vi "Write Scalar Data.vi"(8 "error in (no error)":errorcluster, 9 "Changed?":bool[](array[boolean]), 10 "Values":dbl[](array[numeric]), 11 "Cluster":T1={"Name"="", "Data Type"=enum."<Null>", "session"=0, "Scalar Type"=enum."Standard", "Index"=0, "Length"=0, "attributes"=variant(refnum<k20> refnum), "default value"=variant(refnum<k20> refnum), "RegisterOffset"=0} {"Data Type" format="%.0x"}) -> (0 "error out":errorcluster, 2 "Values":dbl[](array[numeric]))   [LabVIEW 2020, in "FPGA Addon Engine.lvlib"]
uses:
  FPGA Addon Engine.lvlib
  APIs/FPGA Register IO/FPGA Register IO.lvlib
  3b4273db-2eef-454f-a9d7-15a0de1766a4.vi
  da3bfa8f-65e5-4f9a-8452-ca9305b9cf8c.vi
  e9b7ddae-4913-4a74-863a-ac6ad604f706.vi
  60e5d900-6671-49dd-bad3-679abba4dde3.vi
  4f31f09a-b0d0-4122-a737-4d514c13b382.vi
  857dc57c-d282-49ae-bb9f-12b46c14a078.vi
  77a28002-65ef-4437-82ec-1e91d7167048.vi
  660156fa-3609-4cbc-a785-e17faca41079.vi
  <vilib>/fxp/LVFixedPointRepRangeTypeDef.ctl
  <vilib>/fxp/LVFixedPointRepBitsTypeDef.ctl
  APIs/FPGA Register IO/TypeDefs/FXP Configuration.ctl
  Submodules/Source/Types/PWM.Measure.Digital.Settings.ctl
  Submodules/Source/Types/PWM.Measure.Analog.Settings.ctl
  Submodules/Source/Types/WSS.Generate.Digital.Settings.ctl
  Submodules/Source/Types/Sine.Generate.Settings.ctl
  Submodules/Source/Types/Static.Measure.Digital.Settings.ctl
  Submodules/Source/Types/Static.Generate.Digital.Settings.ctl
  Submodules/Source/Types/QuadratureEncoder.Measure.Digital.Settings.ctl
  Submodules/Source/Types/PWM.Generate.Digital.Settings.ctl
  APIs/FPGA Register IO/Write Methods/Write Data Register/Instances/Write SGL.vi
  APIs/FPGA Register IO/Write Methods/Write Data Register/Instances/Write U64.vi
  APIs/FPGA Register IO/Write Methods/Write Data Register/Instances/Write I32.vi
  APIs/FPGA Register IO/Write Methods/Write Data Register/Instances/Write I64.vi
  APIs/FPGA Register IO/Write Methods/Write Data Register/Instances/Write I16.vi
  APIs/FPGA Register IO/Write Methods/Write Data Register/Instances/Write U16.vi
  APIs/FPGA Register IO/Write Methods/Write Data Register/Instances/Write Boolean.vi
  APIs/FPGA Register IO/Write Methods/Write Data Register/Instances/Write FXP.vi
  APIs/FPGA Register IO/Write Methods/Write Data Register/Instances/Write I8.vi
  APIs/FPGA Register IO/Write Methods/Write Data Register/Instances/Write U8.vi
  APIs/FPGA Register IO/Write Methods/Write Data Register/Instances/Write U32.vi
  Types/Register Settings.ctl
  Addon Shared/Types/Scalar Type.ctl
  Addon Shared/FPGA Addon Shared.lvlib
  Addon Shared/Types/FPGA Addon Data Type.ctl
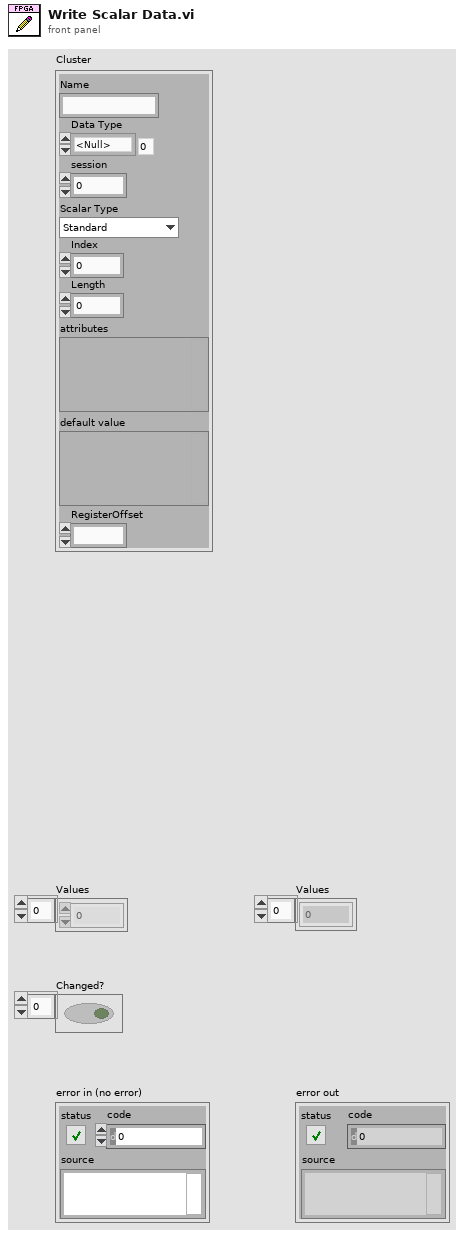
[diagram p1: front panel]
types:
  T1 = typedef "FPGA Addon Engine.lvlib/Register Settings.ctl" = cluster{"Name":string, "Data Type":T2, "session":u32, "Scalar Type":T3, "Index":i32, "Length":i32, "attributes":variant, "default value":variant, "RegisterOffset":u32}
  T2 = typedef "FPGA Addon Shared.lvlib/FPGA Addon Data Type.ctl" = enum8{"<Null>", "I8", "I16", "I32", "I64", "U8", "U16", "U32", "U64", "SGL", "Boolean", "Analog PWM In Settings", "Analog PWM In", "Digital PWM In Settings", "Digital PWM In", "Digital PWM Out", "Sine Out", "FXP", "FXP+/-24.5", "FXP+/-16.5", "FXP+/-32.8", "FXP+/-64.32", "FXP+/-16.7", "FXP+/-20.5", "FXP+/-27.5", "FXP+/-32.16", "FXP+16.3", "FXP+18.3", "Digital Static In", "Digital Static Out", "Digital Static In Settings", "Digital WSS Out", "Quad Encoder Settings", "Quad Encoder In", "Group"}
  T3 = typedef "FPGA Addon Shared.lvlib/Scalar Type.ctl" = enum16{"Standard", "Bitpacked"}
  T4 = typedef "FPGA Register IO.lvlib/FXP Configuration.ctl" = cluster{"FXP Representation":T5, "FXP Range":T6}
  T5 = typedef "LVFixedPointRepBitsTypeDef.ctl" = cluster{"Signed":bool, "Word Length":u32, "Integer Word Length":i32}
  T6 = typedef "LVFixedPointRepRangeTypeDef.ctl" = cluster{"Range Min":dbl, "Range Max":dbl, "Delta":dbl}
  T7 = typedef "Speciality FPGA IO.lvlib/PWM.Measure.Analog.Settings.ctl" = cluster{"ACTIVE EDGE":bool, "TIMEOUT":u32, "THRESHOLD":fxp<+/-,32,8>}
  T8 = typedef "Speciality FPGA IO.lvlib/PWM.Measure.Digital.Settings.ctl" = cluster{"ACTIVE EDGE":bool, "TIMEOUT":u32}
  T9 = typedef "Speciality FPGA IO.lvlib/WSS.Generate.Digital.Settings.ctl" = cluster{"ACTIVE EDGE":bool, "ACTIVE TICKS":u32, "INACTIVE TICKS":u32, "DATA":u8, "SENSOR TYPE":u8}
  T10 = typedef "Speciality FPGA IO.lvlib/Sine.Generate.Settings.ctl" = cluster{"AMP":fxp<+/-,32,8>, "OFFSET":fxp<+/-,32,8>, "PERIODS/TICKS":fxp<+,32,0>}
  T11 = typedef "Speciality FPGA IO.lvlib/Static.Measure.Digital.Settings.ctl" = cluster{"ACTIVE EDGE":bool}
  T12 = typedef "Speciality FPGA IO.lvlib/Static.Generate.Digital.Settings.ctl" = cluster{"ACTIVE EDGE":bool, "OUTPUT":bool}
  T13 = typedef "Speciality FPGA IO.lvlib/QuadratureEncoder.Measure.Digital.Settings.ctl" = cluster{"DIRECTION":u8, "RESET VALUE":i32, "A RESET STATE":bool, "B RESET STATE":bool, "Z RESET STATE":bool}
  T14 = typedef "Speciality FPGA IO.lvlib/PWM.Generate.Digital.Settings.ctl" = cluster{"ACTIVE EDGE":bool, "ACTIVE TICKS":u32, "INACTIVE TICKS":u32}
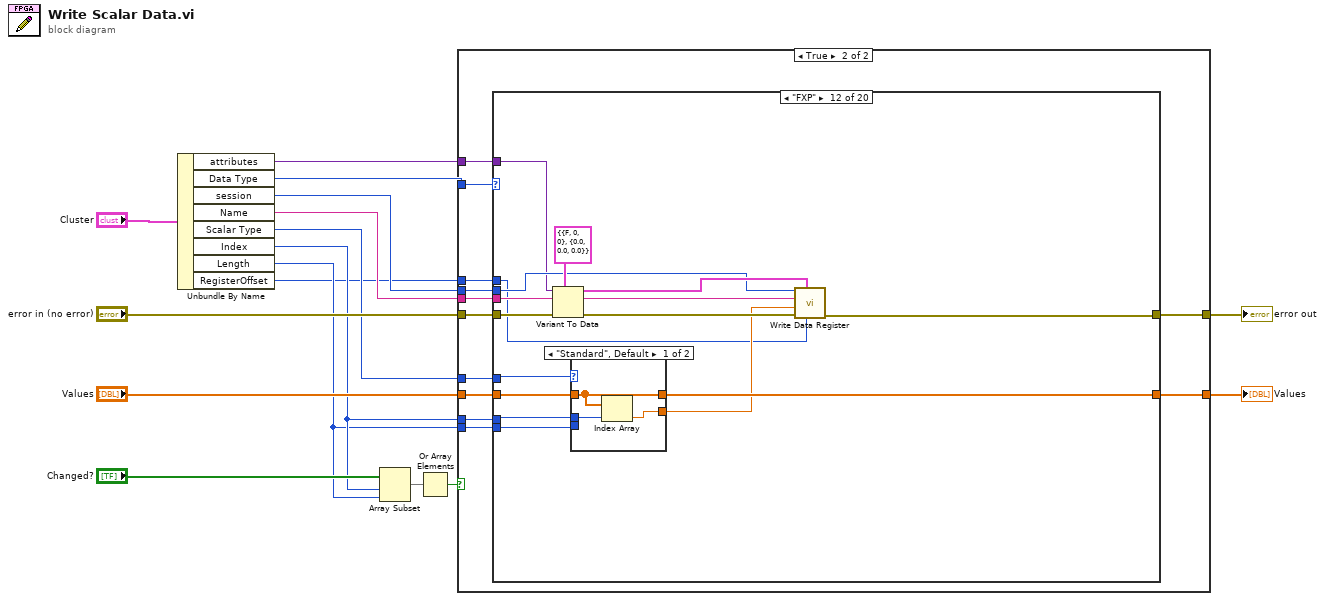
[diagram p0: block diagram]
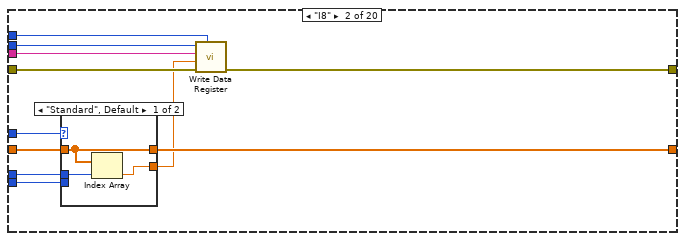
[diagram p4: hidden frame]
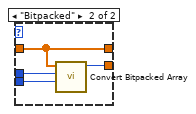
[diagram p5: hidden frame]
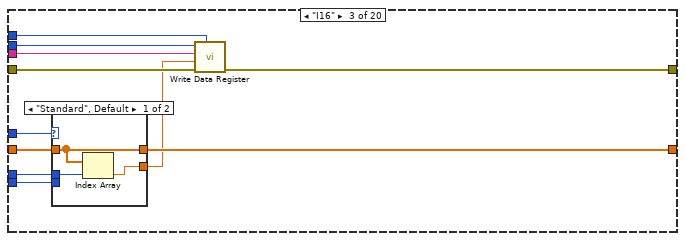
[diagram p6: hidden frame]
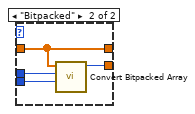
[diagram p7: hidden frame]
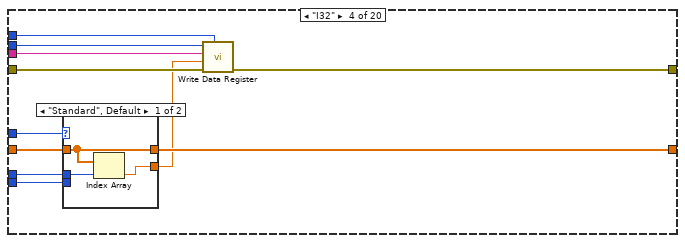
[diagram p8: hidden frame]
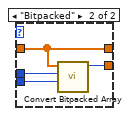
[diagram p9: hidden frame]
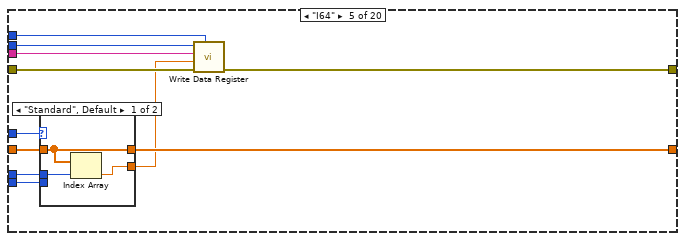
[diagram p10: hidden frame]
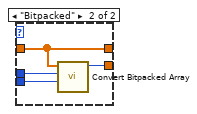
[diagram p11: hidden frame]
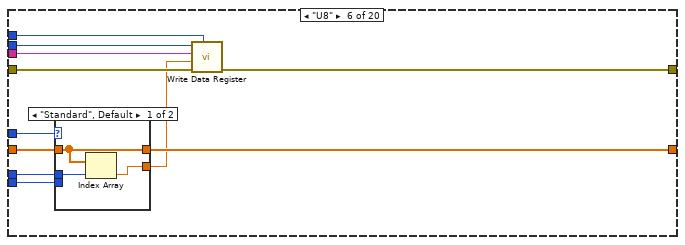
[diagram p12: hidden frame]
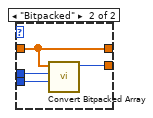
[diagram p13: hidden frame]
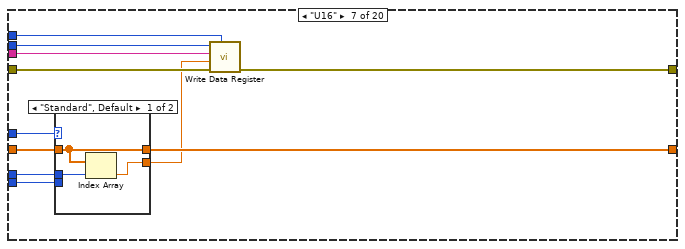
[diagram p14: hidden frame]
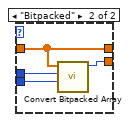
[diagram p15: hidden frame]
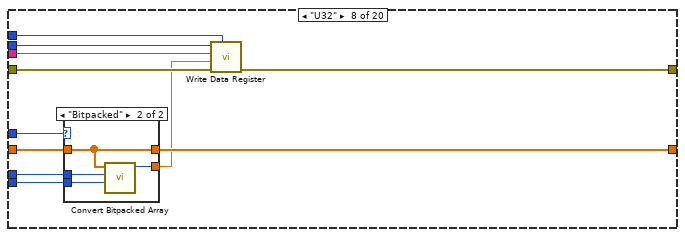
[diagram p16: hidden frame]
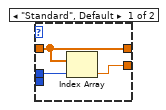
[diagram p17: hidden frame]
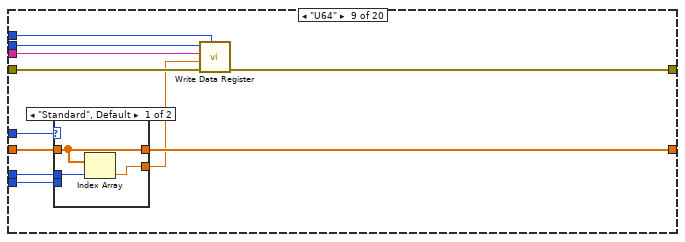
[diagram p18: hidden frame]
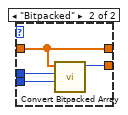
[diagram p19: hidden frame]
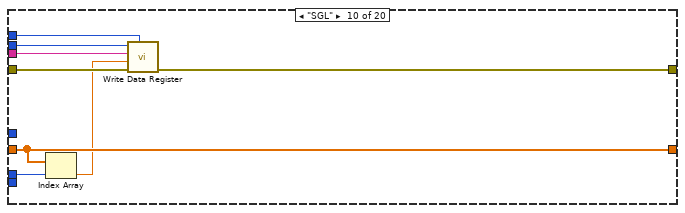
[diagram p20: hidden frame]
diagram:
  n1 = Unbundle By Name("Cluster") -> ("attributes"=w3:variant, "Data Type"=w10:T2, "session"=w7:u32, "Name"=w8:string, "Scalar Type"=w9:T3, "Index"=w6:i32, "Length"=w5:i32, "RegisterOffset"=w1:u32)
  n2 = Array Subset(array="Changed?", index=w6, length=w5) -> (w11:bool[])
  n3 = Or Array Elements(Boolean array=w11) -> (logical OR=w2:bool)
  n4 = case shown="True" w2 {
    tunnel: "error in (no error)" -> [w18 w30]
    tunnel: [w18 w29] -> w15
    tunnel: [w17 w28] -> w14
    tunnel: "Values" -> [w17 w27]
    tunnel: w9 -> [_ w26]
    tunnel: w5 -> [_ w25]
    tunnel: w6 -> [_ w22]
    tunnel: w10 -> [_ w24]
    tunnel: w8 -> [_ w23]
    tunnel: w7 -> [_ w21]
    tunnel: w3 -> [_ w20]
    tunnel: w1 -> [_ w19]
    frame False {
    }
    frame True {
      n5 = case shown="\"FXP\"" w24 {
        tunnel: w30 -> [w32 w40 w57 w74 w92 w112 w129 w147 w166 w182 w190 w208 w221 w237 w251 w275 w290 w304 w318 w337]
        tunnel: [w32 w39 w58 w75 w94 w111 w130 w148 w165 w183 w191 w202 w222 w233 w250 w274 w289 w298 w317 w336] -> w29
        tunnel: [w31 w41 w59 w76 w95 w113 w131 w149 w167 w184 w193 w199 w225 w239 w253 w277 w291 w306 w320 w338] -> w28
        tunnel: w27 -> [w31 w43 w61 w79 w97 w115 w133 w151 w169 w184 w193 w200 w225 w239 w253 w277 w291 w306 w320 w338]
        tunnel: w26 -> [_ w42 w60 w78 w96 w114 w132 w150 w168 _ _ w201 _ _ _ _ _ _ _ _]
        tunnel: w25 -> [_ w35 w53 w77 w89 w107 w125 w143 w161 _ _ w197 w224 w240 w254 w278 w293 w307 w321 w341]
        tunnel: w23 -> [_ w38 w56 w72 w93 w110 w128 w146 w164 w181 w189 w204 w219 w236 w249 w273 w287 w300 w314 w334]
        tunnel: w22 -> [_ w36 w54 w71 w90 w108 w126 w144 w162 w179 w188 w198 w223 w238 w252 w276 w292 w305 w319 w342]
        tunnel: w21 -> [_ w34 w52 w70 w88 w106 w124 w142 w160 w178 w187 w205 w218 w235 w248 w272 w288 w303 w315 w335]
        tunnel: w20 -> [_ _ _ _ _ _ _ _ _ _ _ w203 _ _ _ _ _ _ _ _]
        tunnel: w19 -> [_ w33 w51 w69 w87 w105 w123 w141 w159 w177 w185 w195 _ _ _ _ _ _ _ _]
        frame "<Null>", Default {
        }
        frame "I8" {
          n6 = case shown="\"Standard\", Default" w42 {
            tunnel: w43 -> [w45 w49]
            tunnel: [w46 w50] -> w37
            tunnel: [w45 w49] -> w41
            tunnel: w36 -> [w44 w48]
            tunnel: w35 -> [_ w47]
            frame "Standard", Default {
              n7 = Index Array(array=w45, index=w44) -> (element=w46:dbl)
            }
            frame "Bitpacked" {
              n8 = call "Convert Bitpacked Array.vi"("Length"=w47, "Index"=w48, "Values"=w49) -> ("Numeric"=w50:u64)  [unwired: 8 in]
            }
          }
          n9 = call-poly "Write Data Register.vi"("RegisterOffset"=w33, "error in"=w40, "value in"=w37, "register name"=w38, "session in"=w34) -> ("error out"=w39:errorcluster)  [unwired: 5 in, 1 out]
        }
        frame "I16" {
          n10 = case shown="\"Standard\", Default" w60 {
            tunnel: w61 -> [w63 w67]
            tunnel: [w64 w68] -> w55
            tunnel: [w63 w67] -> w59
            tunnel: w54 -> [w62 w66]
            tunnel: w53 -> [_ w65]
            frame "Standard", Default {
              n11 = Index Array(array=w63, index=w62) -> (element=w64:dbl)
            }
            frame "Bitpacked" {
              n12 = call "Convert Bitpacked Array.vi"("Length"=w65, "Index"=w66, "Values"=w67) -> ("Numeric"=w68:u64)  [unwired: 8 in]
            }
          }
          n13 = call-poly "Write Data Register.vi"("RegisterOffset"=w51, "error in"=w57, "value in"=w55, "register name"=w56, "session in"=w52) -> ("error out"=w58:errorcluster)  [unwired: 5 in, 1 out]
        }
        frame "I32" {
          n14 = case shown="\"Standard\", Default" w78 {
            tunnel: w79 -> [w81 w85]
            tunnel: w77 -> [_ w83]
            tunnel: [w82 w86] -> w73
            tunnel: [w81 w85] -> w76
            tunnel: w71 -> [w80 w84]
            frame "Standard", Default {
              n15 = Index Array(array=w81, index=w80) -> (element=w82:dbl)
            }
            frame "Bitpacked" {
              n16 = call "Convert Bitpacked Array.vi"("Length"=w83, "Index"=w84, "Values"=w85) -> ("Numeric"=w86:u64)  [unwired: 8 in]
            }
          }
          n17 = call-poly "Write Data Register.vi"("RegisterOffset"=w69, "error in"=w74, "value in"=w73, "register name"=w72, "session in"=w70) -> ("error out"=w75:errorcluster)  [unwired: 5 in, 1 out]
        }
        frame "I64" {
          n18 = case shown="\"Standard\", Default" w96 {
            tunnel: w97 -> [w99 w103]
            tunnel: [w100 w104] -> w91
            tunnel: [w99 w103] -> w95
            tunnel: w90 -> [w98 w102]
            tunnel: w89 -> [_ w101]
            frame "Standard", Default {
              n19 = Index Array(array=w99, index=w98) -> (element=w100:dbl)
            }
            frame "Bitpacked" {
              n20 = call "Convert Bitpacked Array.vi"("Length"=w101, "Index"=w102, "Values"=w103) -> ("Numeric"=w104:u64)  [unwired: 8 in]
            }
          }
          n21 = call-poly "Write Data Register.vi"("RegisterOffset"=w87, "error in"=w92, "value in"=w91, "register name"=w93, "session in"=w88) -> ("error out"=w94:errorcluster)  [unwired: 5 in, 1 out]
        }
        frame "U8" {
          n22 = case shown="\"Standard\", Default" w114 {
            tunnel: w115 -> [w117 w121]
            tunnel: [w118 w122] -> w109
            tunnel: [w117 w121] -> w113
            tunnel: w108 -> [w116 w120]
            tunnel: w107 -> [_ w119]
            frame "Standard", Default {
              n23 = Index Array(array=w117, index=w116) -> (element=w118:dbl)
            }
            frame "Bitpacked" {
              n24 = call "Convert Bitpacked Array.vi"("Length"=w119, "Index"=w120, "Values"=w121) -> ("Numeric"=w122:u64)  [unwired: 8 in]
            }
          }
          n25 = call-poly "Write Data Register.vi"("RegisterOffset"=w105, "error in"=w112, "value in"=w109, "register name"=w110, "session in"=w106) -> ("error out"=w111:errorcluster)  [unwired: 5 in, 1 out]
        }
        frame "U16" {
          n26 = case shown="\"Standard\", Default" w132 {
            tunnel: w133 -> [w135 w139]
            tunnel: [w136 w140] -> w127
            tunnel: [w135 w139] -> w131
            tunnel: w126 -> [w134 w138]
            tunnel: w125 -> [_ w137]
            frame "Standard", Default {
              n27 = Index Array(array=w135, index=w134) -> (element=w136:dbl)
            }
            frame "Bitpacked" {
              n28 = call "Convert Bitpacked Array.vi"("Length"=w137, "Index"=w138, "Values"=w139) -> ("Numeric"=w140:u64)  [unwired: 8 in]
            }
          }
          n29 = call-poly "Write Data Register.vi"("RegisterOffset"=w123, "error in"=w129, "value in"=w127, "register name"=w128, "session in"=w124) -> ("error out"=w130:errorcluster)  [unwired: 5 in, 1 out]
        }
        frame "U32" {
          n30 = case shown="\"Bitpacked\"" w150 {
            tunnel: w151 -> [w153 w157]
            tunnel: [w154 w158] -> w145
            tunnel: [w153 w157] -> w149
            tunnel: w144 -> [w152 w156]
            tunnel: w143 -> [_ w155]
            frame "Standard", Default {
              n31 = Index Array(array=w153, index=w152) -> (element=w154:dbl)
            }
            frame "Bitpacked" {
              n32 = call "Convert Bitpacked Array.vi"("Length"=w155, "Index"=w156, "Values"=w157) -> ("Numeric"=w158:u64)  [unwired: 8 in]
            }
          }
          n33 = call-poly "Write Data Register.vi"("RegisterOffset"=w141, "error in"=w147, "value in"=w145, "register name"=w146, "session in"=w142) -> ("error out"=w148:errorcluster)  [unwired: 5 in, 1 out]
        }
        frame "U64" {
          n34 = case shown="\"Standard\", Default" w168 {
            tunnel: w169 -> [w171 w175]
            tunnel: [w172 w176] -> w163
            tunnel: [w171 w175] -> w167
            tunnel: w162 -> [w170 w174]
            tunnel: w161 -> [_ w173]
            frame "Standard", Default {
              n35 = Index Array(array=w171, index=w170) -> (element=w172:dbl)
            }
            frame "Bitpacked" {
              n36 = call "Convert Bitpacked Array.vi"("Length"=w173, "Index"=w174, "Values"=w175) -> ("Numeric"=w176:u64)  [unwired: 8 in]
            }
          }
          n37 = call-poly "Write Data Register.vi"("RegisterOffset"=w159, "error in"=w166, "value in"=w163, "register name"=w164, "session in"=w160) -> ("error out"=w165:errorcluster)  [unwired: 5 in, 1 out]
        }
        frame "SGL" {
          n38 = Index Array(array=w184, index=w179) -> (element=w180:dbl)
          n39 = call-poly "Write Data Register.vi"("RegisterOffset"=w177, "error in"=w182, "value in"=w180, "register name"=w181, "session in"=w178) -> ("error out"=w183:errorcluster)  [unwired: 5 in, 1 out]
        }
        frame "Boolean" {
          n40 = Index Array(array=w193, index=w188) -> (element=w192:dbl)
          n41 = To Unsigned Byte Integer(number=w192) -> (unsigned 8bit integer=w194:u8)
          n42 = Greater Than 0?(x=w194) -> (x > 0?=w186:bool)
          n43 = call-poly "Write Data Register.vi"("RegisterOffset"=w185, "error in"=w190, "value in"=w186, "register name"=w189, "session in"=w187) -> ("error out"=w191:errorcluster)  [unwired: 5 in, 1 out]
        }
        frame "FXP" {
          n44 = Variant To Data(error in=w208, type=T4 {"FXP Representation"={"Signed"=FALSE, "Word Length"=0, "Integer Word Length"=0}, "FXP Range"={"Range Min"=0.0, "Range Max"=0.0, "Delta"=0.0}} ("FXP Configuration"), Variant=w203) -> (data=w206:T4, error out=w207:errorcluster)
          n45 = case shown="\"Standard\", Default" w201 {
            tunnel: w200 -> [w211 w215]
            tunnel: w197 -> [_ w213]
            tunnel: [w212 w216] -> w196
            tunnel: [w211 w215] -> w199
            tunnel: w198 -> [w210 w214]
            frame "Standard", Default {
              n46 = Index Array(array=w211, index=w210) -> (element=w212:dbl)
            }
            frame "Bitpacked" {
              n47 = call "Convert Bitpacked Array.vi"("Length"=w213, "Index"=w214, "Values"=w215) -> ("Numeric"=w216:u64)  [unwired: 8 in]
            }
          }
          n48 = call-poly "Write Data Register.vi"("RegisterOffset"=w195, "FXP Configuration"=w206, "error in"=w207, "DBL Value"=w196, "register name"=w204, "session in"=w205) -> ("error out"=w202:errorcluster)  [unwired: 4 in, 1 out]
        }
        frame "Analog PWM In Settings" {
          n49 = Array Subset(array=w225, index=w223, length=w224) -> (w231:dbl[])
          n50 = Index Array(array=w231) -> (element #1=w229:dbl, element #2=w227:dbl, element #3=w226:dbl)  [unwired: 4 in, 1 out]
          n51 = Greater?(x=w229, y=0.5) -> (0:w228:bool)
          n52 = Bundle By Name(cluster=T7 {"ACTIVE EDGE"=FALSE, "TIMEOUT"=0, "THRESHOLD"=0.0}, "ACTIVE EDGE"=w228, "TIMEOUT"=w227, "THRESHOLD"=w226) -> (w220:T7)
          n53 = call "Write Cluster Register.vim"("error in (no error)"=w221, "Cluster in"=w220, "Cluster Name"=w219, "session in"=w218) -> ("error out"=w222:errorcluster)  [unwired: 6 in, 1 out]
        }
        frame "Digital PWM In Settings" {
          n54 = Array Subset(array=w239, index=w238, length=w240) -> (w245:dbl[])
          n55 = Index Array(array=w245) -> (element #1=w242:dbl, element #2=w241:dbl)  [unwired: 2 in]
          n56 = Greater?(x=w242, y=0.5) -> (0:w244:bool)
          n57 = Bundle By Name(cluster=T8 {"ACTIVE EDGE"=FALSE, "TIMEOUT"=0}, "ACTIVE EDGE"=w244, "TIMEOUT"=w241) -> (w232:T8)
          n58 = call "Write Cluster Register.vim"("error in (no error)"=w237, "Cluster in"=w232, "Cluster Name"=w236, "session in"=w235) -> ("error out"=w233:errorcluster)  [unwired: 6 in, 1 out]
        }
        frame "Digital WSS Out" {
          # "Speed\nData\nPPR\nWD\nSensor"
          n59 = Array Subset(array=w253, index=w252, length=w254) -> (w269:dbl[])
          n60 = Index Array(array=w269) -> (element #1=w267:dbl, element #2=w266:dbl, element #3=w265:dbl, element #4=w264:dbl, element #5=w263:dbl)  [unwired: 5 in]
          n61 = Absolute Value(x=w267) -> (abs(x)=w255:dbl)
          n62 = To Single Precision Float(number=w264) -> (single precision float=w258:sgl)
          n63 = To Single Precision Float(number=w255) -> (single precision float=w260:sgl)
          n64 = To Single Precision Float(number=w265) -> (single precision float=w259:sgl)
          n65 = call "WSS_Data_Conversion.vi"("WD"=w258, "PPR"=w259, "Speed"=w260) -> ("Inactive"=w256:u32, "Active"=w257:u32)  [unwired: 7 in]
          n66 = To Unsigned Byte Integer(number=w266) -> (unsigned 8bit integer=w261:u8)
          n67 = To Unsigned Byte Integer(number=w263) -> (unsigned 8bit integer=w262:u8)
          n68 = Bundle By Name(cluster=T9 {"ACTIVE EDGE"=FALSE, "ACTIVE TICKS"=0, "INACTIVE TICKS"=0, "DATA"=0, "SENSOR TYPE"=0} ("Settings"), "ACTIVE EDGE"=TRUE, "ACTIVE TICKS"=w257, "INACTIVE TICKS"=w256, "DATA"=w261, "SENSOR TYPE"=w262) -> (w247:T9)
          n69 = call "Write Cluster Register.vim"("error in (no error)"=w251, "Cluster in"=w247, "Cluster Name"=w249, "session in"=w248) -> ("error out"=w250:errorcluster)  [unwired: 6 in, 1 out]
        }
        frame "Sine Out" {
          n70 = Array Subset(array=w277, index=w276, length=w278) -> (w284:dbl[])
          n71 = Index Array(array=w284) -> (element #1=w280:dbl, element #2=w281:dbl, element #3=w282:dbl)  [unwired: 3 in]
          n72 = Divide(x=w282, y=sgl 40000000.0) -> (x/y=w279:dbl)
          n73 = Bundle By Name(cluster=T10 {"AMP"=0.0, "OFFSET"=0.0, "PERIODS/TICKS"=0.0} ("Settings"), "AMP"=w280, "OFFSET"=w281, "PERIODS/TICKS"=w279) -> (w271:T10)
          n74 = call "Write Cluster Register.vim"("error in (no error)"=w275, "Cluster in"=w271, "Cluster Name"=w273, "session in"=w272) -> ("error out"=w274:errorcluster)  [unwired: 6 in, 1 out]
        }
        frame "Digital Static In Settings" {
          n75 = Array Subset(array=w291, index=w292, length=w293) -> (w294:dbl[])
          n76 = Index Array(array=w294) -> (element=w297:dbl)  [unwired: 1 in]
          n77 = Greater?(x=w297, y=0.5) -> (0:w295:bool)
          n78 = Bundle By Name(cluster=T11 {"ACTIVE EDGE"=FALSE} ("Settings"), "ACTIVE EDGE"=w295) -> (w286:T11)
          n79 = call "Write Cluster Register.vim"("error in (no error)"=w290, "Cluster in"=w286, "Cluster Name"=w287, "session in"=w288) -> ("error out"=w289:errorcluster)  [unwired: 6 in, 1 out]
        }
        frame "Digital Static Out" {
          w310 = 0.5 ("y")
          n80 = Array Subset(array=w306, index=w305, length=w307) -> (w312:dbl[])
          n81 = Index Array(array=w312) -> (element #1=w311:dbl, element #2=w309:dbl)  [unwired: 2 in]
          n82 = Greater?(x=w311, y=w310) -> (0:w308:bool)
          n83 = Greater?(x=w309, y=w310) -> (0:w299:bool)
          n84 = Bundle By Name(cluster=T12 {"ACTIVE EDGE"=FALSE, "OUTPUT"=FALSE} ("Settings"), "ACTIVE EDGE"=w308, "OUTPUT"=w299) -> (w302:T12)
          n85 = call "Write Cluster Register.vim"("error in (no error)"=w304, "Cluster in"=w302, "Cluster Name"=w300, "session in"=w303) -> ("error out"=w298:errorcluster)  [unwired: 6 in, 1 out]
        }
        frame "Quad Encoder Settings" {
          w325 = 0.5 ("y")
          n86 = Array Subset(array=w320, index=w319, length=w321) -> (w331:dbl[])
          n87 = Index Array(array=w331) -> (element #1=w322:dbl, element #2=w323:dbl, element #3=w326:dbl, element #4=w327:dbl, element #5=w328:dbl)  [unwired: 5 in]
          n88 = Greater?(x=w326, y=w325) -> (0:w324:bool)
          n89 = Greater?(x=w327, y=w325) -> (0:w329:bool)
          n90 = Greater?(x=w328, y=w325) -> (0:w330:bool)
          n91 = Bundle By Name(cluster=T13 {"DIRECTION"=0, "RESET VALUE"=0, "A RESET STATE"=FALSE, "B RESET STATE"=FALSE, "Z RESET STATE"=FALSE} ("Settings"), "DIRECTION"=w322, "RESET VALUE"=w323, "A RESET STATE"=w324, "B RESET STATE"=w329, "Z RESET STATE"=w330) -> (w316:T13)
          n92 = call "Write Cluster Register.vim"("error in (no error)"=w318, "Cluster in"=w316, "Cluster Name"=w314, "session in"=w315) -> ("error out"=w317:errorcluster)  [unwired: 6 in, 1 out]
        }
        frame "Digital PWM Out" {
          n93 = Array Subset(array=w338, index=w342, length=w341) -> (w358:dbl[])
          n94 = Index Array(array=w358) -> (element #1=w355:dbl, element #2=w353:dbl, element #3=w354:dbl)  [unwired: 3 in]
          n95 = To Single Precision Float(number=w354) -> (single precision float=w346:sgl)
          n96 = To Single Precision Float(number=w353) -> (single precision float=w347:sgl)
          n97 = In Range and Coerce(upper limit=sgl 100.0, x=w346, lower limit=sgl 0.0) -> (coerced(x)=w345:sgl)  [unwired: 1 out]
          n98 = Equal To 0?(x=w347) -> (x = 0?=w352:bool)
          n99 = Divide(x=sgl 40000000.0 ("y"), y=w347) -> (x/y=w350:sgl)
          n100 = Multiply(x=w345, y=sgl 0.01 ("x")) -> (x*y=w348:sgl)
          n101 = case shown="False" w352 {
            tunnel: [w363 w364] -> w351
            tunnel: w350 -> [w363 _]
            tunnel: [w362 w364] -> w349
            tunnel: w348 -> [w362 _]
            frame False {
            }
            frame True {
              w364 = sgl 0.0
            }
          }
          n102 = Greater?(x=w355, y=0.5) -> (0:w356:bool)
          n103 = To Unsigned Long Integer(number=w351) -> (unsigned 32bit integer=w360:u32)
          n104 = Multiply(x=w351, y=w349) -> (x*y=w339:u32)
          n105 = Subtract(x=w360, y=w339) -> (x-y=w340:u32)
          n106 = Bundle By Name(cluster=T14 {"ACTIVE EDGE"=FALSE, "ACTIVE TICKS"=0, "INACTIVE TICKS"=0} ("Settings"), "ACTIVE EDGE"=w356, "INACTIVE TICKS"=w340, "ACTIVE TICKS"=w339) -> (w333:T14)
          n107 = call "Write Cluster Register.vim"("error in (no error)"=w337, "Cluster in"=w333, "Cluster Name"=w334, "session in"=w335) -> ("error out"=w336:errorcluster)  [unwired: 6 in, 1 out]
        }
      }
    }
  }
  "error out" <- w15
  "Values" <- w14
